vi "Bridge_Release_Lease.vi"(8 "error in (no error)":errorcluster={"status"=FALSE, "code"=0, "source"="\"\""}, 10 "release reason":string, 11 "Lease token":string) -> (0 "error out":errorcluster={"status"=FALSE, "code"=0, "source"="\"\""}, 2 "status ok":bool, 3 "Release ACK":string)   [LabVIEW 2026]
doc: "INTENT: Return resource ownership. LOGIC: Release only matching token; log final status; do not reassign while old commands active."
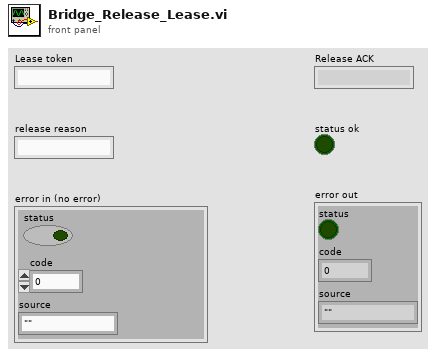
[diagram p1: front panel]
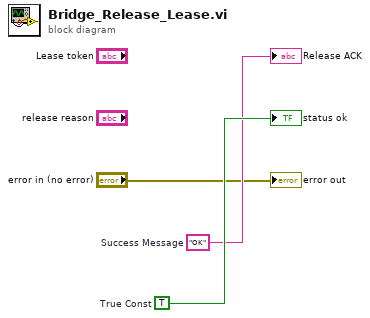
[diagram p0: block diagram]
diagram:
  w3 = TRUE  # True Const
  w2 = "OK"  # Success Message
  "Release ACK" <- w2
  "status ok" <- w3
  "error out" <- "error in (no error)"
